vi "Daily Yield.vi"() -> ()   [LabVIEW 2026]
uses:
  <vilib>/addons/database/Connection.llb/DB Tools Open Connec (String).vi
  <vilib>/addons/database/Connection.llb/Conn Execute.vi
  <vilib>/addons/database/Recordset.llb/Rec Fetch Recordset Data (R).vi
  <vilib>/addons/database/Recordset.llb/Rec Destroy - Connection.vi
  <vilib>/addons/database/_DB Variant To Data/Database Variant To Data.xnode
  <vilib>/addons/database/NI_Database_API.lvlib
panel:
  out "Daily Yield":string[][](table)
  in  "error in (no error)":errorcluster
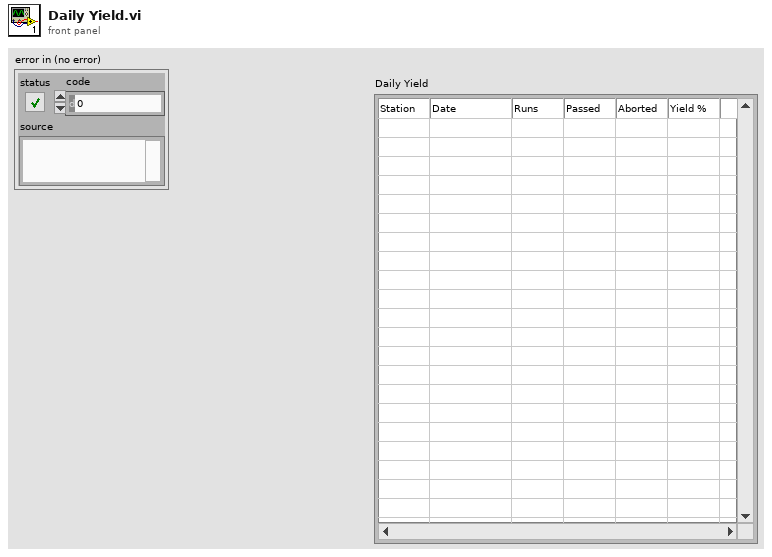
[diagram p1: front panel]
types:
  T1 = typedef "NI_Database_API.lvlib/Conn ObjectReference.ctl" = refnum<k1>
  T2 = typedef "NI_Database_API.lvlib/Rec ObjectReference.ctl" = refnum<k1>
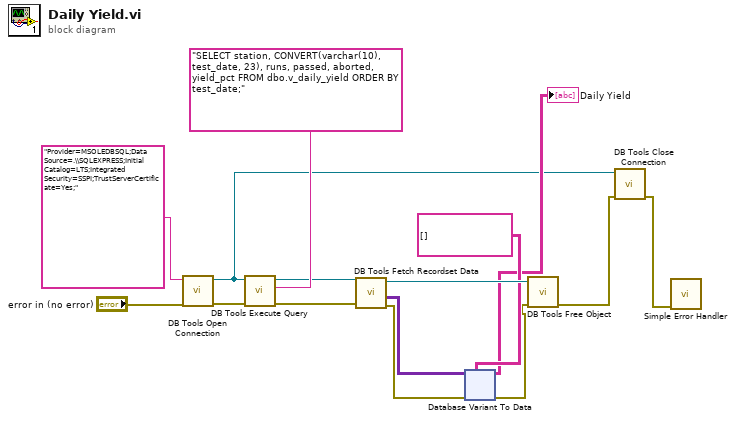
[diagram p0: block diagram]
diagram:
  n1 = call-poly <vilib>:"DB Tools Open Connection.vi"("error in (no error)"="error in (no error)", "connection information"="Provider=MSOLEDBSQL;Data Source=.\\SQLEXPRESS;Initial Catalog=LTS;Integrated Security=SSPI;TrustServerCertificate=Yes;") -> ("error out"=w11:errorcluster, "connection reference"=w3:T1)  [unwired: 6 in]
  n2 = call-poly <vilib>:"DB Tools Execute Query.vi"("error in (no error)"=w11, "SQL query"="SELECT station, CONVERT(varchar(10), test_date, 23), runs, passed, aborted, yield_pct FROM dbo.v_daily_yield ORDER BY test_date;", "connection reference"=w3) -> ("error out"=w10:errorcluster, "recordset reference"=w13:T2)  [unwired: 5 in]
  n3 = call-poly <vilib>:"DB Tools Fetch Recordset Data.vi"("error in (no error)"=w10, "recordset reference"=w13) -> ("error out"=w7:errorcluster, "recordset data"=w5:variant[][], "recordset reference out"=w12:T2)  [unwired: 3 in]
  n4 = xnode "Database Variant To Data"("database variant"=w5, "error in (no error)"=w7, "type"=string[][] []) -> ("data"=→"Daily Yield":string[][], "error out"=w6:errorcluster)
  n5 = call-poly <vilib>:"DB Tools Free Object.vi"("error in (no error)"=w6, "recordset reference"=w12) -> ("error out"=w2:errorcluster)  [unwired: 8 in, 1 out]
  n6 = call <vilib>:"DB Tools Close Connection.vi"("error in (no error)"=w2, "connection reference"=w3) -> ("error out"=w1:errorcluster)  [unwired: 5 in]
  n7 = call <vilib>:"Simple Error Handler.vi"("error in (no error)"=w1) -> ()  [unwired: 4 in, 5 out]
